vi "JsonRpcResponseClusterToToolReturn.vi"(8 "error in (no error)":errorcluster, 10 "JsonRPCHttpResponseBody":T1) -> (0 "error out":errorcluster, 2 "ToolReturn":cluster{"id":string, "result":variant})   [LabVIEW 2017]
uses:
  <vilib>/LVH/i3 JSON/JSON Generation/Create Value Files/Create Value - Object.vi
  <vilib>/LVH/i3 JSON/JSON Generation/Add Object Parameter Files/Add Object Parameter - Numeric.vi
  <vilib>/LVH/i3 JSON/JSON Generation/Add Object Parameter Files/Add Object Parameter - String.vi
  <vilib>/LVH/i3 JSON/i3-json.lvlib
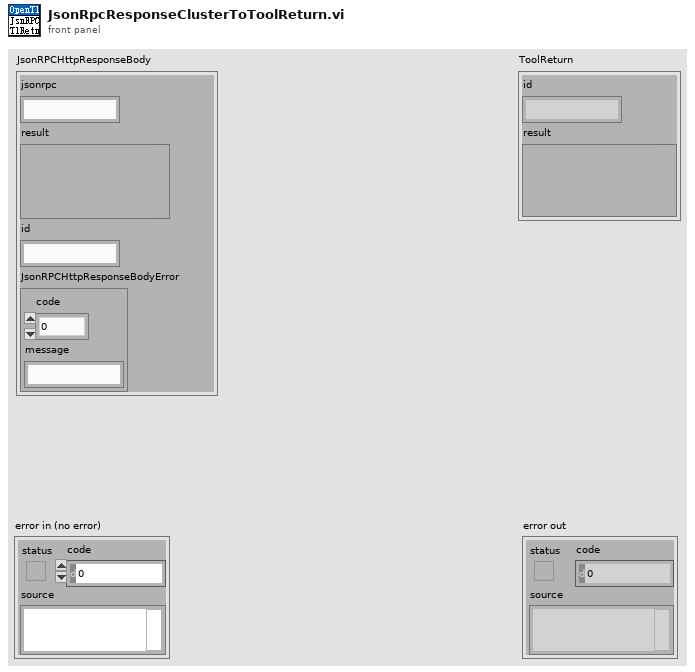
[diagram p1: front panel]
types:
  T1 = cluster{"jsonrpc":string, "result":variant, "id":string, "JsonRPCHttpResponseBodyError":cluster{"code":i32, "message":string}}
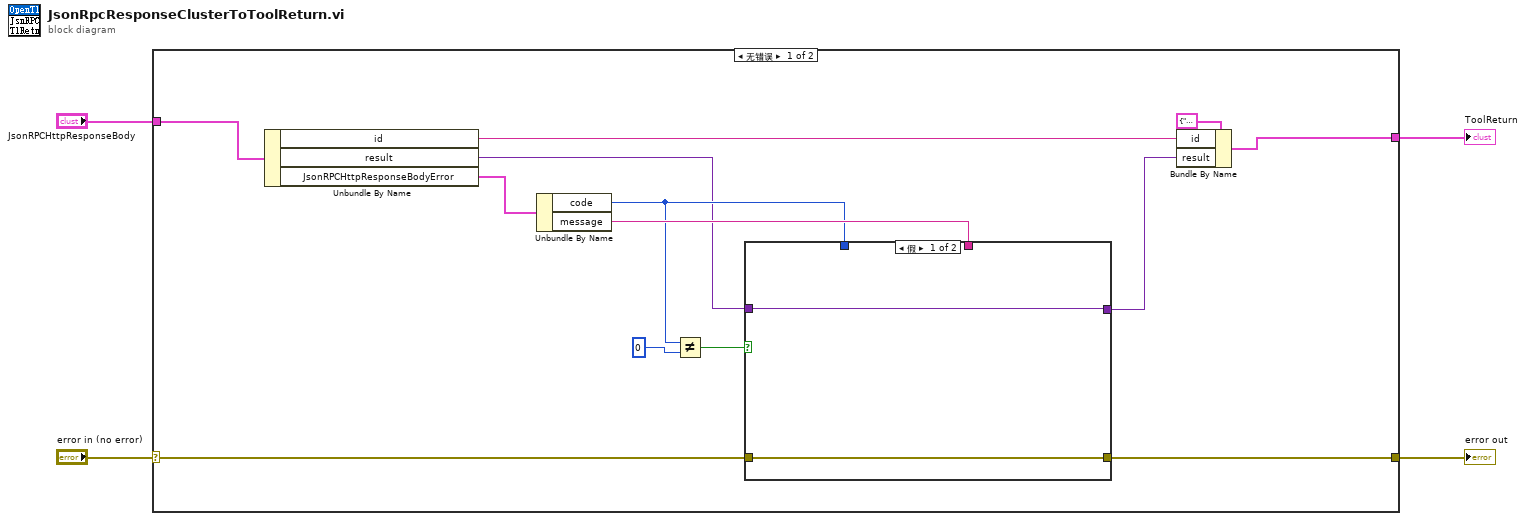
[diagram p0: block diagram]
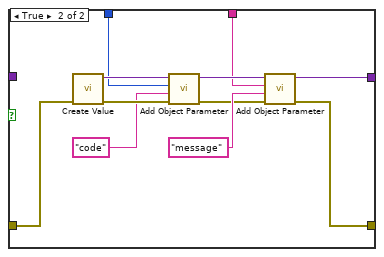
[diagram p2: hidden frame]
diagram:
  n1 = case shown="无错误" "error in (no error)" {
    selector: "error in (no error)" -> [w7 w31]
    tunnel: [w6 w31] -> w3
    tunnel: "JsonRPCHttpResponseBody" -> [w17 _]
    tunnel: [w5 _] -> w1
    frame No Error {
      n2 = Unbundle By Name(w17) -> ("id"=w15:string, "result"=w9:variant, "JsonRPCHttpResponseBodyError"=w14:cluster{"code":i32, "message":string})
      n3 = Unbundle By Name(w14) -> ("code"=w12:i32, "message"=w13:string)
      n4 = Not Equal?(x=w12, y=0) -> (x != y?=w10:bool)
      n5 = case shown="假" w10 {
        tunnel: w13 -> [_ w26]
        tunnel: w12 -> [_ w23]
        tunnel: w9 -> [w19 _]
        tunnel: [w19 w22] -> w8
        tunnel: w7 -> [w18 w21]
        tunnel: [w18 w20] -> w6
        frame False {
        }
        frame True {
          n6 = call-poly <vilib>:"Create Value.vi"("error in (no error)"=w21) -> ("error out"=w28:errorcluster, "JSON Tree"=w30:variant)  [unwired: 9 in]
          n7 = call-poly <vilib>:"Add Object Parameter.vi"("error in (no error)"=w28, "Name"="code" ("id"), "Numeric"=w23, "JSON Tree in (JSON Object)"=w30) -> ("error out"=w24:errorcluster, "JSON Tree out (JSON Object)"=w29:variant)  [unwired: 6 in]
          n8 = call-poly <vilib>:"Add Object Parameter.vi"("error in (no error)"=w24, "Name"="message" ("id"), "String"=w26, "JSON Tree in (JSON Object)"=w29) -> ("error out"=w20:errorcluster, "JSON Tree out (JSON Object)"=w22:variant)  [unwired: 6 in]
        }
      }
      n9 = Bundle By Name(cluster=cluster{"id":string, "result":variant} {"id"="", "result"=variant} ("ToolReturn"), "id"=w15, "result"=w8) -> (w5:cluster{"id":string, "result":variant})
    }
    frame Error {
    }
  }
  "error out" <- w3
  "ToolReturn" <- w1
